vi "UMLEditor_PackageClasses.vi"(0 "DiagramIn":refnum<class "Graph.lvclass">, 3 "Settings":T1={"Levels"=-1}, 5 "error in (no error)":errorcluster) -> (19 "error out":errorcluster)   [LabVIEW 2020]
doc: "Gets current diagram values"
uses:
  <resource>/Framework/Providers/Open_GDS/UML/UMLEditor/UMLEditor_PackageClasses.ctl
  <resource>/Framework/Providers/Open_GDS/UML/Graph_class/Graph.lvclass
  <resource>/Framework/Providers/Open_GDS/UML/Graphics_class/FontType.ctl
  <resource>/Framework/Providers/Open_GDS/UML/UMLEditor/UMLEditor BusyDialogAction.ctl
  <resource>/Framework/Providers/Open_GDS/UML/ClassNode_class/ClassNode.lvclass
  C:/Program Files (x86)/National Instruments/LabVIEW 2020/resource/Framework/Providers/Open_GDS/UML/AbstractNode_class/AbstractNode.lvclass
  <resource>/Framework/Providers/Open_GDS/UML/PackageNode_class/PackageNode.lvclass
  C:/Program Files (x86)/National Instruments/LabVIEW 2020/resource/Framework/Providers/Open_GDS/UML/RectangularNode_class/RectangularNode.lvclass
  <resource>/Framework/Providers/Open_GDS/UML/ContextHelp/ContextHelp_HelpTexts.ctl
  <resource>/Framework/Providers/Open_GDS/UML/General/Point/Point Point2D.ctl
  <resource>/Framework/Providers/Open_GDS/UML/RectangularNode_class/RectangularNode.lvclass
  <resource>/Framework/Providers/Open_GDS/UML/Graphics_class/Graphics.lvclass
  <resource>/Framework/Providers/Open_GDS/UML/AbstractNode_class/AbstractNode.lvclass
panel:
  in  "MoveNodes":bool
  in  "Levels":i32=3 caption="Maximum levels of packages to create" min=1 max=100
  in  "Help":bool
  in  "cancel":bool
  in  "ok":bool
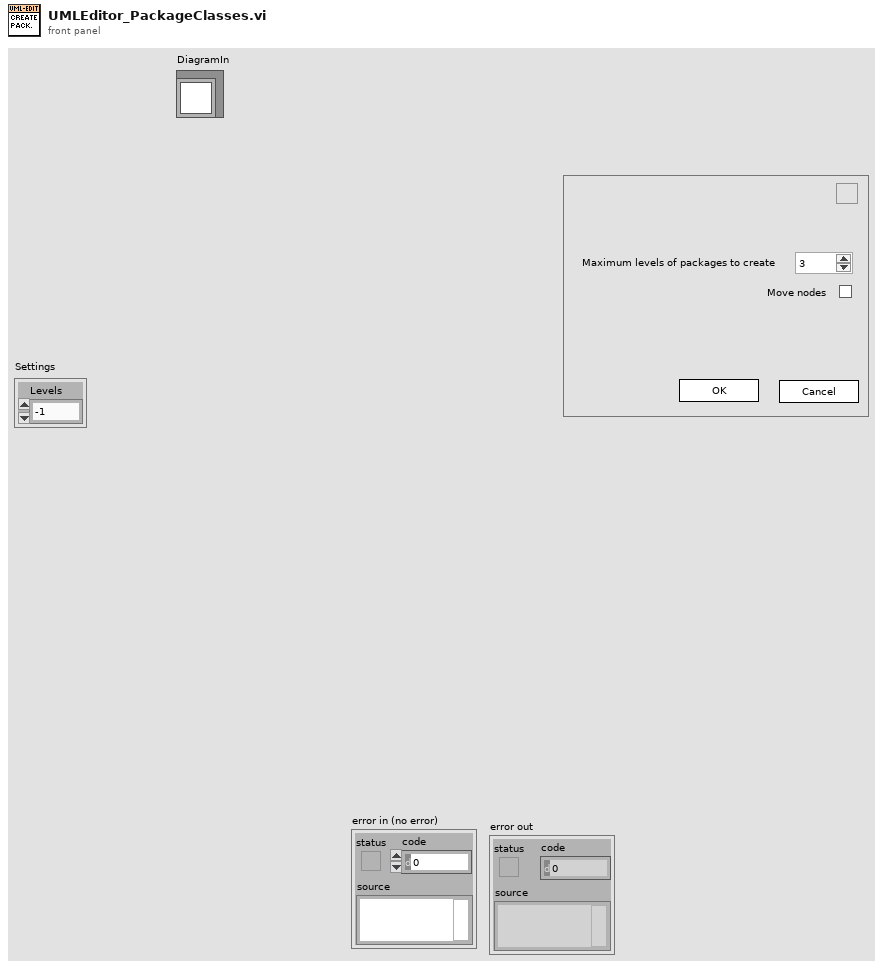
[diagram p1: front panel]
types:
  T1 = typedef "UMLEditor_PackageClasses.ctl" = cluster{"Levels":i32}
  T2 = cluster{"ClassNodes":refnum<class "ClassNode.lvclass">[], "Folders":cluster{"Foldername":string, "Path":path, "Nodes":refnum<class "ClassNode.lvclass">[], "SubFolders":path[], "PackageNode":refnum<class "PackageNode.lvclass">}[], "PackageNames":string[], "PackagesNodes":refnum<class "PackageNode.lvclass">[]}
  T3 = typedef "UMLEditor BusyDialogAction.ctl" = enum16{"Initialize", "Open(VIs)", "Open(i)", "Send_I-Value", "SendStatusMessage", "GetBusyDialogStatus", "Close", "Quit"}
  T4 = typedef "Graphics.lvclass/FontType.ctl" = cluster{"Font Name:":string, "Size":i16, "Strikeout?":bool, "Italic?":bool, "Underline?":bool, "Outline?":bool, "Shadow?":bool, "Bold?":bool}
  T5 = typedef "ContextHelp_HelpTexts.ctl" = enum16{"None(Hide)", "Default", "Help", "Welcome", "GettingStarted", "ClassDiagram_Help", "SequenceDiagram_Help", "UseCaseDiagram_Help", "BSelect", "BClass", "BInterface", "BPackage", "BNote", "BDependency", "BInheritance", "BInterfaceImplementation", "BAssociation", "BAggregation", "BCompAggregation", "BNoteConnector", "BObject", "BActionBar", "BCall", "BSystem", "BActor", "BUseCase", "BGeneralization", "BIncludes", "BExtends", "BUseCaseDiagramAssociation", "ClassRelationshipEdge editDialog_Bent Style", "ClassRelationshipEdge editDialog_RelationType", "ClassRelationshipEdge editDialog_Reverse association", "ClassRelationshipEdge editDialog_Start label", "ClassRelationshipEdge editDialog_Middle label", "ClassRelationshipEdge editDialog_End label", "UMLEditor reversedEngineering_Pathes", "ReversedEngineering StateReverseDialog_Help", "ReversedEngineering StateQueuedSettings_Help", "UMLEditor reversedEngineering_AddTopVIs", "UMLEditor reversedEngineering_AddClasses", "UMLEditor reversedEngineering_AddDirs", "UMLEditor reversedEngineering_Recursively", "UMLEditor reversedEngineering_Remove", "UMLEditor reversedEngineering_ClearList", "UMLEditor reversedEngineering_HideSubAss", "UMLEditor reversedEngineering_CreateTypes", "UMLEditor reversedEngineering_OnlyInheritance", "UMLEditor reversedEngineering_CreateApplication", "UMLEditor reversedEngineering_OK", "UMLEditor reversedEngineering_Cancel", "UMLEditor reversedEngineering_Help", "UMLEditor createWizardScriptFile_ScriptfilePath", "UMLEditor createWizardScriptFile_ClassPath", "UMLEditor createWizardScriptFile_Use", "UMLEditor createWizardScriptFile_PrivateDirName", "UMLEditor createWizardScriptFile_DirAppend", "UMLEditor createWizardScriptFile_Separator Character", "UMLEditor createWizardScriptFile_OK", "UMLEditor createWizardScriptFile_Cancel", "UMLEditor createWizardScriptFile_Help", "ClassNode editDialog_Class Name", "InterfaceNode editDialog_Class Name", "ClassNode editDialog_Attribute", "ClassNode editDialog_Methods", "InterfaceNode editDialog_Methods", "ClassNode editDialog_connection", "InterfaceNode editDialog_connection", "ClassNode editDialog_StereoType", "ClassNode editDialog_ShowAttrib", "ClassNode editDialog_ShowMethods", "ClassNode editDialog_ClassPath", "ClassNode editDialog_AddAttribute", "ClassNode editDialog_AddMethod", "InterfaceNode editDialog_AddMethod", "ClassNode AttributeGuide_AttributeName", "ClassNode AttributeGuide_Array?", "ClassNode AttributeGuide_Data Type", "ClassNode AttributeGuide_RefName", "ClassNode AttributeGuide_Preview", "ClassNode AttributeGuide_OK", "ClassNode AttributeGuide_Cancel", "ClassNode MethodGuide_Visibility", "ClassNode MethodGuide_Method Name", "ClassNode MethodGuide_Preview", "ClassNode MethodGuide_OK", "ClassNode MethodGuide_Cancel", "CallNode EditCallProperties_AllButtons", "ObjectNode EditObjectlProperties_AllButtons", "ActorNode EditActorProperties_AllButtons", "UseCaseRelationshipNode EditUseCaselProperties_AllButtons", "UseCaseNode EditUseCaselProperties_AllButtons", "SystemNode EditSystemProperties_AllButtons", "ReversedEngineering UpdateAttributes_AllButtons", "StateNode editDialog_AllButtons", "StateTransition editDialog_AllButtons", "ArrangeNodes Main_Picture", "ArrangeNodes Main_Zoom", "ArrangeNodes Main_Auto Zoom", "ArrangeNodes Main_shorten", "ArrangeNodes Main_Min Length", "ArrangeNodes Main_Max Length", "ArrangeNodes Main_increase", "ArrangeNodes Main_decrease", "ArrangeNodes Main_Shake", "ArrangeNodes Main", "BState", "BInitialState", "BFinalState", "BStateTransition", "StateDiagram_Help", "StateDiagram_PropertiesAllButtons", "ReversedEngineering StateReverseDialog_ClearStates", "ReversedEngineering StateReverseDialog_UseQueuedStateMachines", "ReversedEngineering StateReverseDialog_QueuedSettings", "ReversedEngineering StateReverseDialog_SearchForVIs", "ReversedEngineering StateReverseDialog_SearchCriteria", "OptionsDialog_ClassBasePath", "OptionsDialog_VIPath", "OptionsDialog_ApplicationPath", "OptionsDialog_WizDir", "OptionsDialog_IniFilePath", "OptionsDialog_DefineColors", "OptionsDialog_Help", "OptionsDialog_CreateTypes", "ClassRelationshipEdge editDialog_SplitWire"}
  T6 = typedef "Point Point2D.ctl" = cluster{"x":dbl, "y":dbl}
  T7 = typedef "ContextHelp_ShowType.ctl" = cluster{"Header":string, "Picture":picture, "Text":string}
  T8 = cluster{"Foldername":string, "Path":path, "Nodes":refnum<class "ClassNode.lvclass">[], "SubFolders":path[], "PackageNode":refnum<class "PackageNode.lvclass">}
  T9 = cluster{"Foldername":string, "Path":path, "Nodes":refnum<class "ClassNode.lvclass">[], "SubFolders":path[], "PackageNode":refnum<class "PackageNode.lvclass">}[]
  T10 = typedef "Rectangle Rectangle2D.ctl" = cluster{"x":dbl, "y":dbl, "width":dbl, "height":dbl}
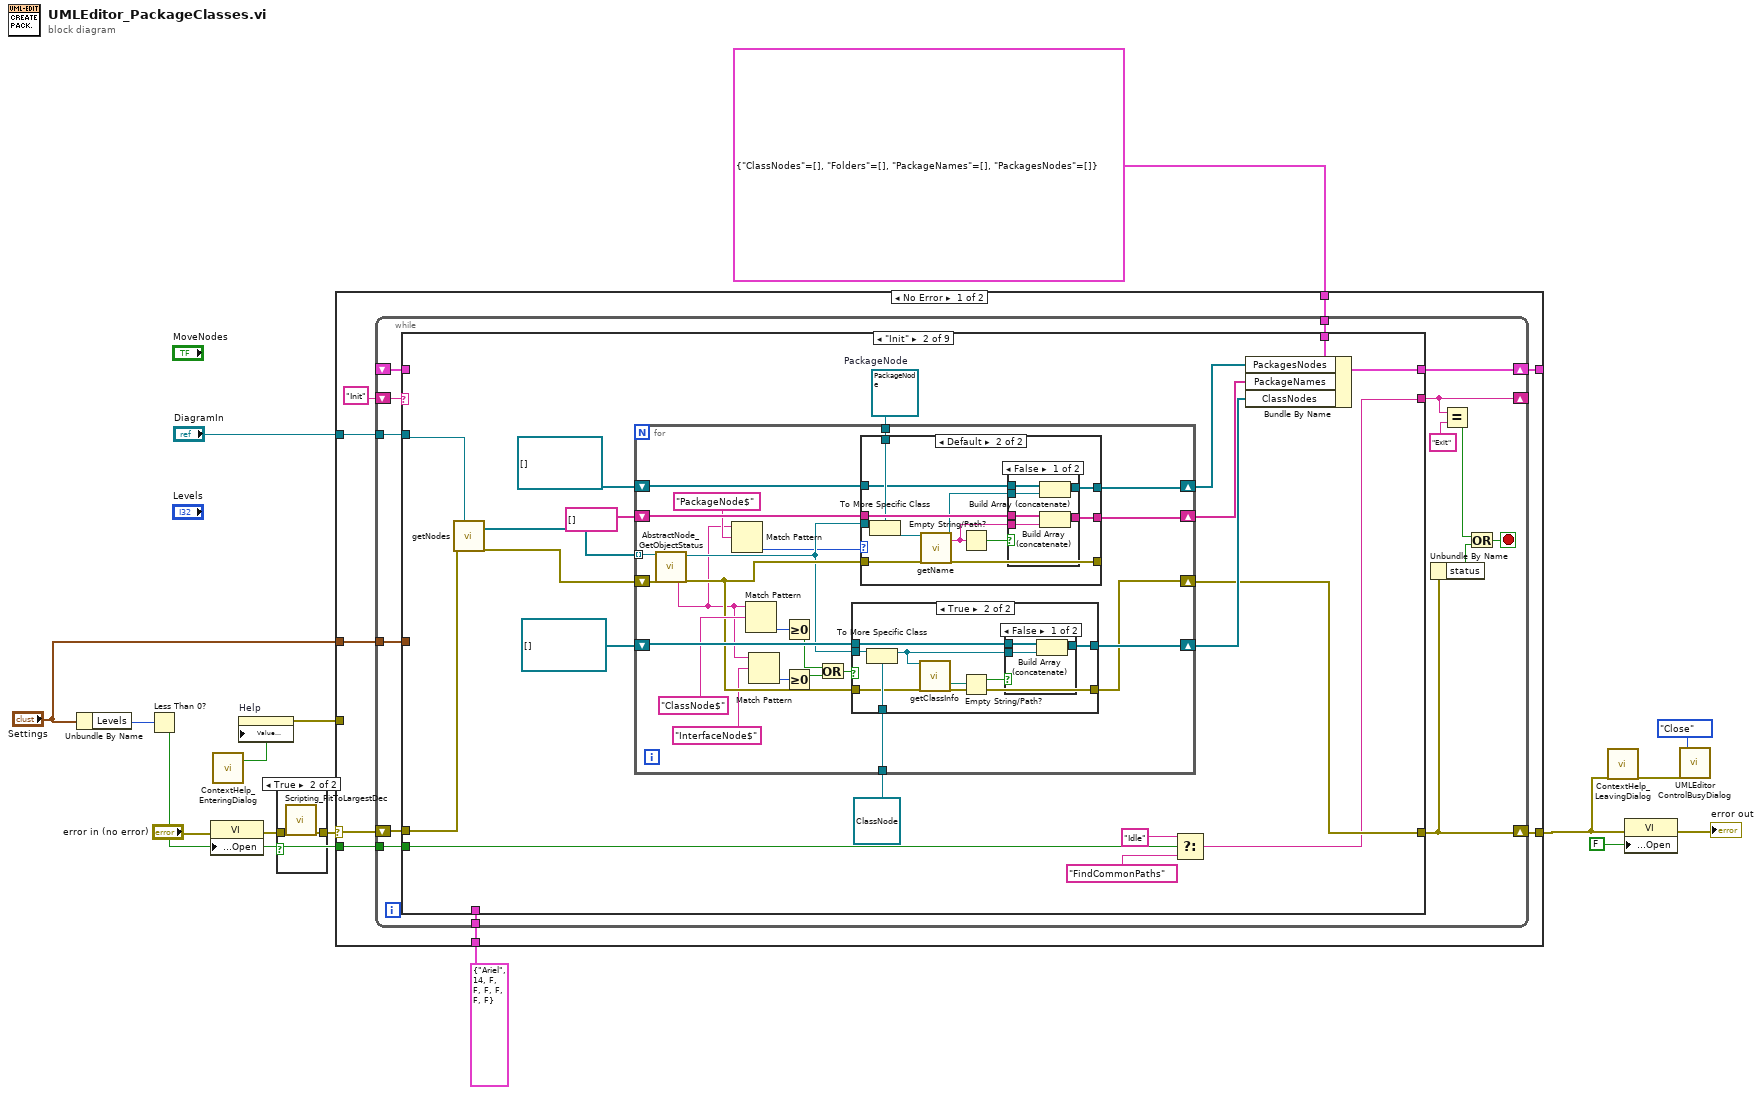
[diagram p0: block diagram]
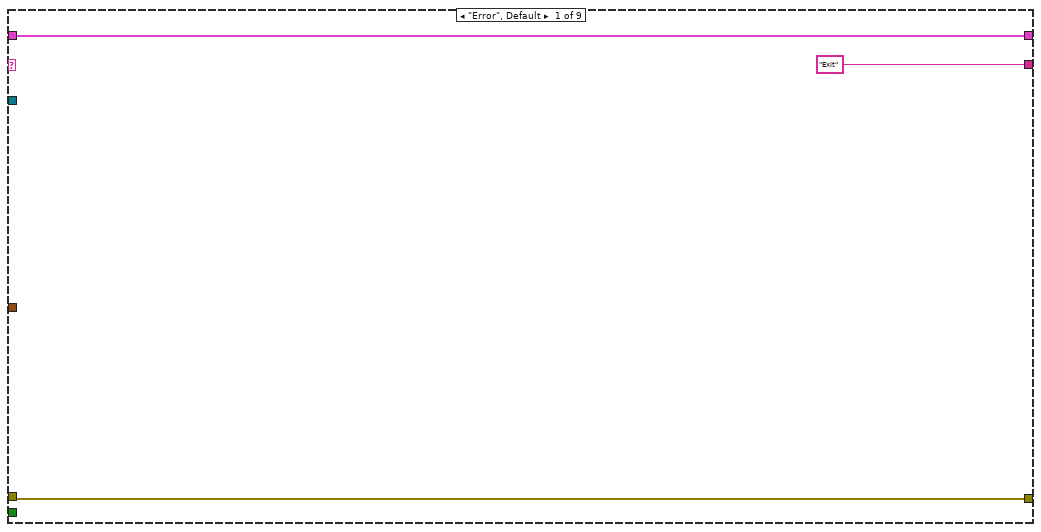
[diagram p3: hidden frame]
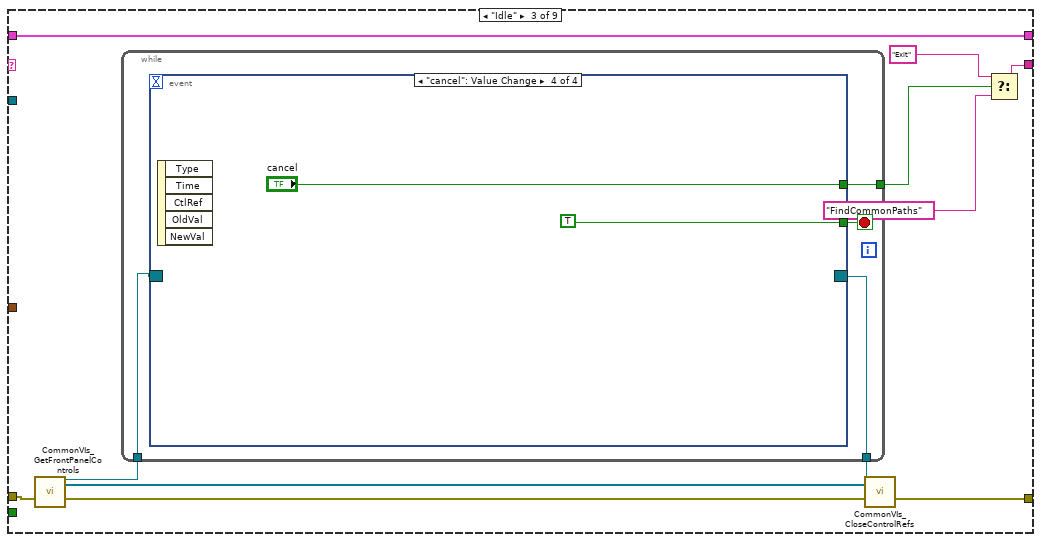
[diagram p8: hidden frame]
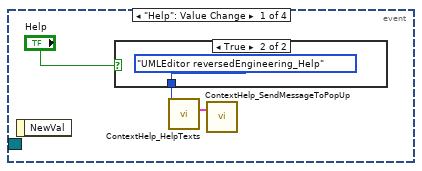
[diagram p9: hidden frame]
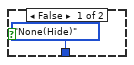
[diagram p10: hidden frame]
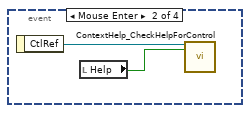
[diagram p11: hidden frame]
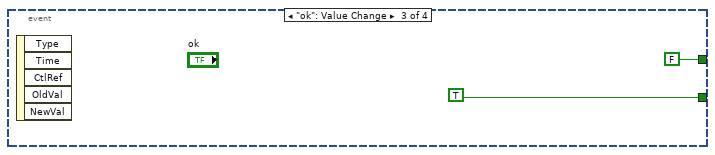
[diagram p12: hidden frame]
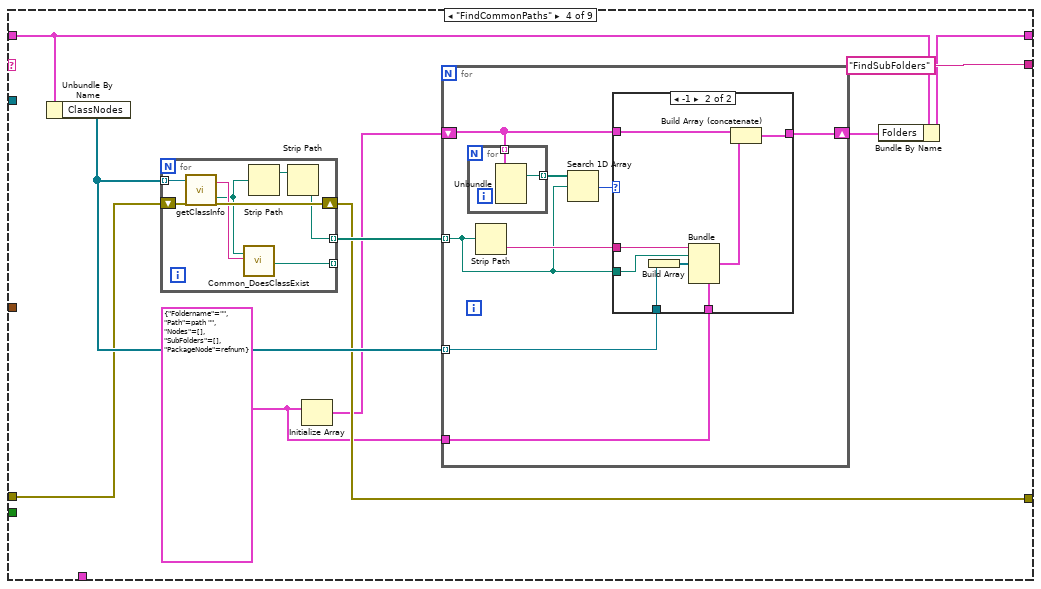
[diagram p13: hidden frame]
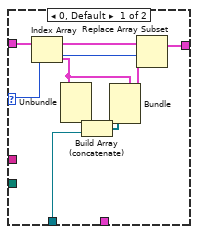
[diagram p14: hidden frame]
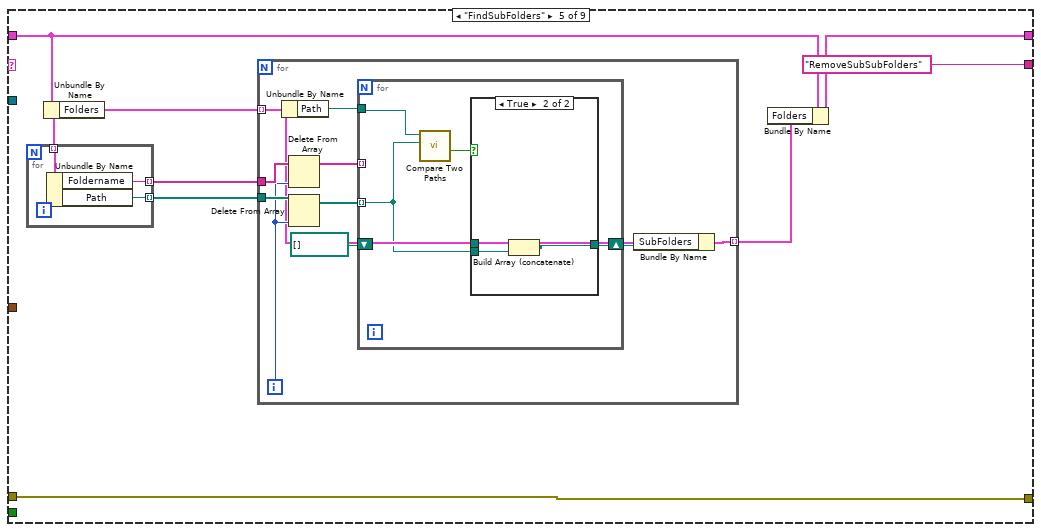
[diagram p15: hidden frame]
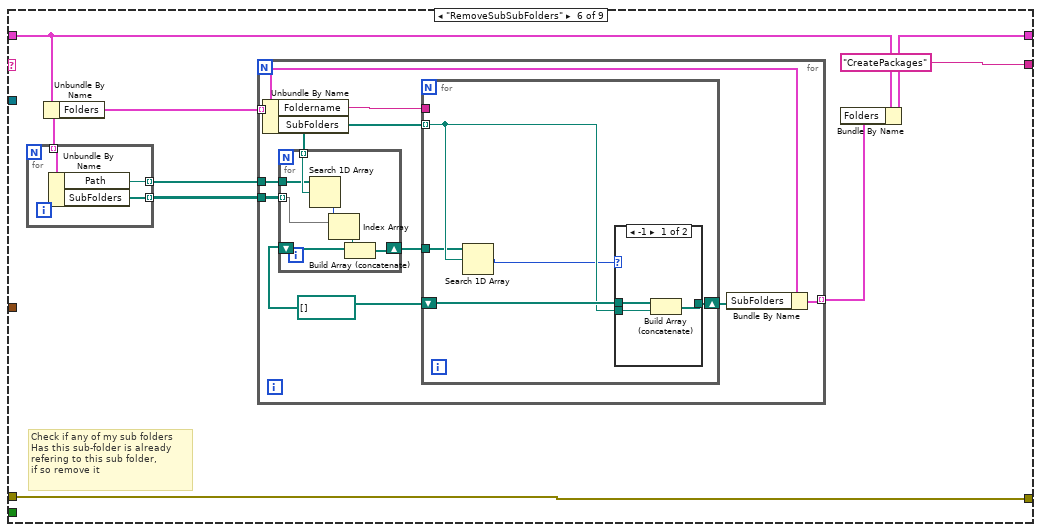
[diagram p17: hidden frame]
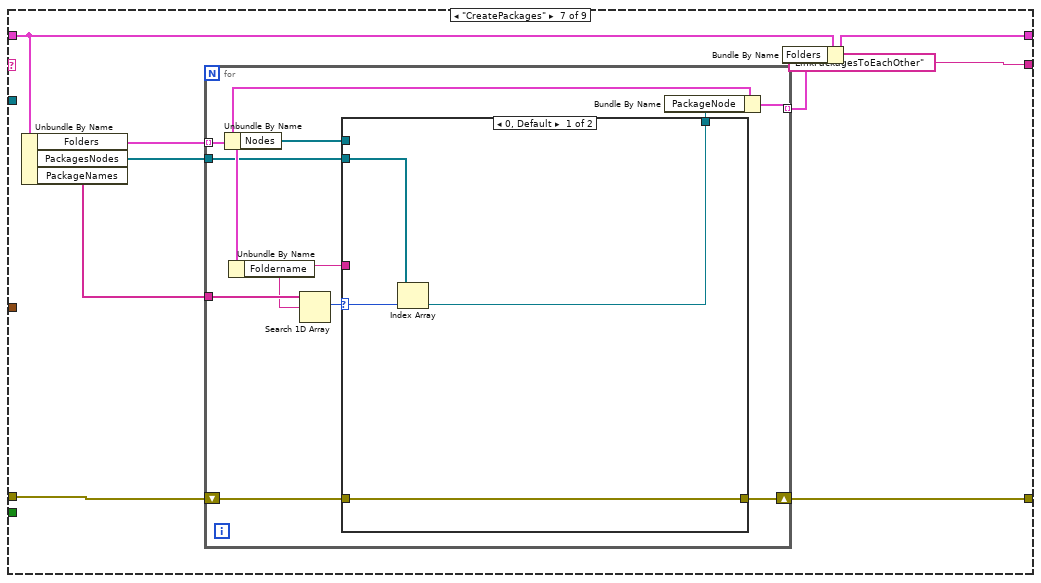
[diagram p19: hidden frame]
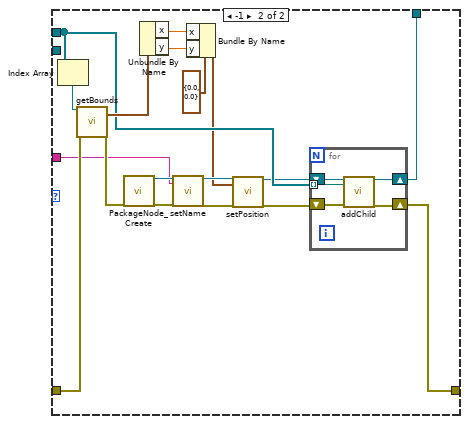
[diagram p20: hidden frame]
diagram:
  n1 = Unbundle By Name("Settings") -> ("Levels"=w5:i32)
  n2 = Less Than 0?(x=w5) -> (x < 0?=w4:bool)
  n3 = property class="VI"(error in="error in (no error)", "Front Panel.Open"=w4) -> (error out=w7:errorcluster)  [unwired: 1 in, 1 out]
  n4 = call <resource>:"ContextHelp_EnteringDialog.vi"() -> ("HelpStatus"=w16:bool)  [unwired: 1 in, 18 out]
  n5 = property on="Help" class="Bool (strict)"("Value (Signaling)"=w16) -> (error out=w15:errorcluster)  [unwired: 2 in, 1 out]
  n6 = case shown="True" w4 {
    tunnel: w7 -> [w17 w19]
    tunnel: [w17 w18] -> w6
    frame False {
    }
    frame True {
      n7 = call <resource>:"Scripting_FitToLargestDec.vi"("error in (no error)"=w19) -> ("error out"=w18:errorcluster)  [unwired: 5 in, 1 out]
    }
  }
  n8 = case shown="No Error" w6 {
    selector: w6 -> [w26 w379]
    tunnel: [w27 w379] -> w12
    tunnel: [w25 _] -> _
    tunnel: w15 -> [_ _]
    tunnel: T4 {"Font Name:"="Ariel", "Size"=14, "Strikeout?"=FALSE, "Italic?"=FALSE, "Underline?"=FALSE, "Outline?"=FALSE, "Shadow?"=FALSE, "Bold?"=FALSE} ("font") -> [w24 _]
    tunnel: w4 -> [w23 _]
    tunnel: T2 {"ClassNodes"=[], "Folders"=[], "PackageNames"=[], "PackagesNodes"=[]} ("local") -> [w22 _]
    tunnel: "Settings" -> [w21 _]
    tunnel: "DiagramIn" -> [w20 _]
    frame No Error {
      n9 = while {
        shift-right: [w40] -> w27
        shift-left: w26 -> [w29]
        shift-right: [w38] -> _
        shift-left: "Init" -> [w43]
        shift-right: [w42] -> w25
        shift-left: _ -> [w41]
        tunnel: w24 -> [w34]
        tunnel: w23 -> [w33]
        tunnel: w22 -> [w32]
        tunnel: w21 -> [w31]
        tunnel: w20 -> [w30]
        stop <- w35 stop-if-true
        n10 = case shown="\"Init\"" w43 {
          tunnel: [w44 w57 w127 w158 w201 w232 w264 w309 w355] -> w40
          tunnel: [w45 w60 w129 w153 w195 w226 w265 w314 w359] -> w42
          tunnel: ["Exit" w53 w134 "FindSubFolders" ("y") "RemoveSubSubFolders" ("y") "CreatePackages" ("y") "LinkPackagesToEachOther" ("y") "AddPackagesToGraph" ("y") "Exit" ("y")] -> w38
          tunnel: w41 -> [w45 _ w129 w154 w196 w227 w266 w314 w359]
          tunnel: w34 -> [_ _ _ _ _ _ _ _ _]
          tunnel: w33 -> [_ w56 _ _ _ _ _ _ _]
          tunnel: w32 -> [_ w61 _ _ _ _ _ _ _]
          tunnel: w31 -> [_ _ _ _ _ _ _ _ _]
          tunnel: w30 -> [_ w62 _ _ _ _ _ _ w360]
          tunnel: w29 -> [w44 w51 w127 w152 w201 w232 w263 w315 w354]
          frame "Error", Default {
          }
          frame "Init" {
            w50 = refnum<class "PackageNode.lvclass"> refnum  # PackageNode
            n11 = call-dynamic "getNodes.vi"("reference"=w62, "error in (no error)"=w51) -> ("nodes"=w59:refnum<class "AbstractNode.lvclass">[], "error out"=w64:errorcluster)  [unwired: 15 in, 1 out]
            n12 = for {
              shift-right: [w82] -> w57
              shift-left: w64 -> [w88]
              tunnel: w59 -> [w87] mode=indexing
              shift-right: [w85] -> w58
              shift-left: refnum<class "ClassNode.lvclass">[] [] -> [w86]
              tunnel: refnum<class "ClassNode.lvclass"> refnum ("reference out") -> [w83]
              shift-right: [w75] -> w49
              shift-left: string[] [] -> [w79]
              tunnel: w50 -> [w81]
              shift-right: [w74] -> w47
              shift-left: refnum<class "PackageNode.lvclass">[] [] -> [w73]
              n13 = call <resource>:"AbstractNode_GetObjectStatus.vi"("reference in"=w87, "error in (no error)"=w88) -> ("Class name"=w72:string, "reference out"=w78:refnum<class "AbstractNode.lvclass">, "error out"=w80:errorcluster)  [unwired: 15 out]
              n14 = Match Pattern(string=w72, regular expression="PackageNode$") -> (offset past match=w76:i32)  [unwired: 4 out]
              n15 = Match Pattern(string=w72, regular expression="ClassNode$") -> (offset past match=w69:i32)  [unwired: 4 out]
              n16 = Match Pattern(string=w72, regular expression="InterfaceNode$") -> (offset past match=w70:i32)  [unwired: 4 out]
              n17 = Greater Or Equal To 0?(x=w69) -> (x >= 0?=w67:bool)
              n18 = Greater Or Equal To 0?(x=w70) -> (x >= 0?=w68:bool)
              n19 = Or(x=w67, y=w68) -> (x .or. y?=w66:bool)
              n20 = case shown="True" w66 {
                tunnel: w86 -> [w113 w122]
                tunnel: w78 -> [_ w120]
                tunnel: [w113 w121] -> w85
                tunnel: w83 -> [_ w119]
                tunnel: w80 -> [w112 w117]
                tunnel: [w112 w114] -> w82
                frame False {
                }
                frame True {
                  n21 = To More Specific Class(target class=w119, reference=w120) -> (specific class reference=w118:refnum<class "ClassNode.lvclass">)  [unwired: 1 in, 1 out]
                  n22 = call-dynamic "getClassInfo.vi"("reference"=w118, "error in (no error)"=w117) -> ("ClassPath"=w116:path, "error out"=w114:errorcluster)  [unwired: 8 in, 8 out]
                  n23 = Empty String/Path?(string/path=w116) -> (empty?=w115:bool)
                  n24 = case shown="False" w115 {
                    tunnel: w122 -> [w125 w126]
                    tunnel: [w124 w126] -> w121
                    tunnel: w118 -> [w123 _]
                    frame False {
                      n25 = Build Array (concatenate)(w125, w123) -> (w124:refnum<class "ClassNode.lvclass">[])
                    }
                    frame True {
                    }
                  }
                }
              }
              n26 = case shown="Default" w76 {
                tunnel: w79 -> [w91 w103]
                tunnel: w78 -> [_ w101]
                tunnel: [w91 w102] -> w75
                tunnel: w80 -> [w90 w97]
                tunnel: [w90 w95] -> _
                tunnel: w81 -> [_ w99]
                tunnel: [w89 w94] -> w74
                tunnel: w73 -> [w89 w93]
                frame -1 {
                }
                frame Default {
                  n27 = To More Specific Class(target class=w99, reference=w101) -> (specific class reference=w98:refnum<class "PackageNode.lvclass">)  [unwired: 1 in, 1 out]
                  n28 = call-dynamic "getName.vi"("reference"=w98, "error in (no error)"=w97) -> ("reference out"=w92:refnum<class "PackageNode.lvclass">, "name"=w96:string, "error out"=w95:errorcluster)  [unwired: 15 in]
                  n29 = Empty String/Path?(string/path=w96) -> (empty?=w100:bool)
                  n30 = case shown="False" w100 {
                    tunnel: w103 -> [w106 w111]
                    tunnel: [w109 w111] -> w102
                    tunnel: w96 -> [w108 _]
                    tunnel: [w107 w110] -> w94
                    tunnel: w93 -> [w105 w110]
                    tunnel: w92 -> [w104 _]
                    frame False {
                      n31 = Build Array (concatenate)(w105, w104) -> (w107:refnum<class "PackageNode.lvclass">[])
                      n32 = Build Array (concatenate)(w106, w108) -> (w109:string[])
                    }
                    frame True {
                    }
                  }
                }
              }
            }
            n33 = Select(t="Idle" ("y"), s=w56, f="FindCommonPaths") -> (s? t:f=w53:string)
            n34 = Bundle By Name(cluster=w61, "PackagesNodes"=w47, "PackageNames"=w49, "ClassNodes"=w58) -> (w60:T2)
          }
          frame "Idle" {
            n35 = call <resource>:"CommonVIs_GetFrontPanelControls.vi"() -> ("Event Registration Refnum"=w132:refnum<event-registration>, "ControlRefs"=w130:refnum<vi>[])  [unwired: 2 in, 16 out]
            n36 = while {
              tunnel: [w139] -> w128
              tunnel: w132 -> [w137]
              tunnel: [w136] -> w131
              stop <- w138 stop-if-true
              n37 = event shown="[3] \"cancel\": Value Change" {
                selector: w137 -> [_ _ _ _]
                dyn-events: [_ _ _ _] -> w136
                timeout: _ -> [_ _ _ _]
                tunnel: [_ _ FALSE ("cancel") "cancel"] -> w139
                tunnel: [_ _ TRUE ("Front Panel Window:Is Frontmost") TRUE ("Front Panel Window:Is Frontmost")] -> w138
                event "Help": Value Change {
                  n38 = event-data() -> ()  [unwired: 2 out]
                  n39 = case shown="True" "Help" {
                    tunnel: [ContextHelp_HelpTexts."None(Hide)" ("HelpText") ContextHelp_HelpTexts."UMLEditor reversedEngineering_Help" ("HelpText")] -> w141
                    frame False {
                    }
                    frame True {
                    }
                  }
                  n40 = call <resource>:"ContextHelp_HelpTexts.vi"("HelpText (enum or string)"=w141) -> ("HelpOut"=w142:T7)  [unwired: 18 out]
                  n41 = call <resource>:"ContextHelp_SendMessageToPopUp.vi"("PopUpMessage"=w142) -> ()  [unwired: 2 in, 17 out]
                }
                event Mouse Enter {
                  n42 = event-data() -> ("CtlRef"=w146:refnum<vi>)  [unwired: 1 out]
                  n43 = local read "Help"() -> (w145:bool)
                  n44 = call <resource>:"ContextHelp_CheckHelpForControl.vi"("Ctl Refnum"=w146, "Help"=w145) -> ()  [unwired: 1 in, 17 out]
                }
                event "ok": Value Change {
                  n45 = event-data() -> ()  [unwired: 6 out]
                }
                event "cancel": Value Change {
                  n46 = event-data() -> ()  [unwired: 6 out]
                }
              }
            }
            n47 = call <resource>:"CommonVIs_CloseControlRefs.vi"("Event Registration Refnum"=w131, "ControlRefs"=w130) -> ()  [unwired: 1 in, 17 out]
            n48 = Select(t="Exit", s=w128, f="FindCommonPaths") -> (s? t:f=w134:string)
          }
          frame "FindCommonPaths" {
            w156 = T8 {"Foldername"="", "Path"=path "", "Nodes"=[], "SubFolders"=[], "PackageNode"=refnum}
            n49 = Unbundle By Name(w154) -> ("ClassNodes"=w160:refnum<class "ClassNode.lvclass">[])
            n50 = for {
              tunnel: w160 -> [w194] mode=indexing
              shift-right: [w192] -> w158
              shift-left: w152 -> [w193]
              tunnel: [w187] -> w159 mode=indexing
              tunnel: [w190] -> _ mode=indexing
              n51 = call-dynamic "getClassInfo.vi"("reference"=w194, "error in (no error)"=w193) -> ("className"=w191:string, "ClassPath"=w188:path, "error out"=w192:errorcluster)  [unwired: 8 in, 7 out]
              n52 = call <resource>:"Common_DoesClassExist.vi"("ClassPath"=w188, "ClassName"=w191) -> ("llb/LvCLass-Path"=w190:path)  [unwired: 17 out]
              n53 = Strip Path(path=w188) -> (stripped path=w189:path)  [unwired: 1 out]
              n54 = Strip Path(path=w189) -> (stripped path=w187:path)  [unwired: 1 out]
            }
            n55 = Initialize Array(w156) -> (w157:T9)  [unwired: 1 in]
            n56 = for {
              tunnel: w159 -> [w161] mode=indexing
              tunnel: w160 -> [w163] mode=indexing
              shift-right: [w168] -> w151
              shift-left: w157 -> [w166]
              tunnel: w156 -> [w162]
              n57 = for {
                tunnel: [w185] -> w167 mode=indexing
                tunnel: w166 -> [w186] mode=indexing
                n58 = Unbundle(w186) -> ("Path"=w185:path)  [unwired: 4 out]
              }
              n59 = Strip Path(path=w161) -> (name=w165:string)  [unwired: 1 out]
              n60 = Search 1D Array(1D array=w167, element=w161) -> (index of element=w164:i32)  [unwired: 1 in]
              n61 = case shown="-1" w164 {
                selector: w164 -> [w173 _]
                tunnel: w161 -> [_ w184]
                tunnel: [w172 w183] -> w168
                tunnel: w166 -> [w174 w182]
                tunnel: w165 -> [_ w181]
                tunnel: w163 -> [w175 w180]
                tunnel: w162 -> [_ w179]
                frame 0, Default {
                  n62 = Index Array(array=w174, index=w173) -> (element=w171:T8)
                  n63 = Unbundle(w171) -> ("Nodes"=w176:refnum<class "ClassNode.lvclass">[])  [unwired: 4 out]
                  n64 = Build Array (concatenate)(w176, w175) -> (w170:refnum<class "ClassNode.lvclass">[])
                  n65 = Bundle(cluster=w171, "Nodes"=w170) -> (w169:T8)  [unwired: 4 in]
                  n66 = Replace Array Subset(array=w174, new element=w169, index=w173) -> (w172:T9)
                }
                frame -1 {
                  n67 = Build Array(w180) -> (w178:refnum<class "ClassNode.lvclass">[])
                  n68 = Bundle(cluster=w179, "Foldername"=w181, "Path"=w184, "Nodes"=w178) -> (w177:T8)  [unwired: 2 in]
                  n69 = Build Array (concatenate)(w182, w177) -> (w183:T9)
                }
              }
            }
            n70 = Bundle By Name(cluster=w154, "Folders"=w151) -> (w153:T2)
          }
          frame "FindSubFolders" {
            n71 = Unbundle By Name(w196) -> ("Folders"=w200:T9)
            n72 = for {
              tunnel: w200 -> [w205] mode=indexing
              tunnel: [w204] -> w198 mode=indexing
              tunnel: [w203] -> w199 mode=indexing
              n73 = Unbundle By Name(w205) -> ("Foldername"=w204:string, "Path"=w203:path)
            }
            n74 = for {
              tunnel: w200 -> [w209] mode=indexing
              tunnel: w199 -> [w215]
              tunnel: w198 -> [w214]
              tunnel: [w207] -> w197 mode=indexing
              i -> [w213]
              n75 = Unbundle By Name(w209) -> ("Path"=w212:path)
              n76 = Delete From Array(array=w214, index=w213) -> (array with subset deleted=w210:string[])  [unwired: 1 in, 1 out]
              n77 = Delete From Array(array=w215, index=w213) -> (array with subset deleted=w211:path[])  [unwired: 1 in, 1 out]
              n78 = for {
                tunnel: w212 -> [w220]
                tunnel: w211 -> [w216] mode=indexing
                shift-right: [w217] -> w208
                shift-left: path[] [] -> [w218]
                tunnel: w210 -> [_] mode=indexing
                n79 = call <vilib>:"Compare Two Paths.vi"("Path 2"=w216, "Path 1"=w220) -> ("Path 2 Relative to Path 1?"=w219:bool)  [unwired: 6 in, 3 out]
                n80 = case shown="True" w219 {
                  tunnel: w218 -> [w221 w224]
                  tunnel: w216 -> [_ w223]
                  tunnel: [w221 w222] -> w217
                  frame False {
                  }
                  frame True {
                    n81 = Build Array (concatenate)(w224, w223) -> (w222:path[])
                  }
                }
              }
              n82 = Bundle By Name(cluster=w209, "SubFolders"=w208) -> (w207:T8)
            }
            n83 = Bundle By Name(cluster=w196, "Folders"=w197) -> (w195:T2)
          }
          frame "RemoveSubSubFolders" {
            # "Check if any of my sub folders\nHas this sub-folder is already \nrefering to this sub folder,\nif so remove it"
            n84 = Unbundle By Name(w227) -> ("Folders"=w231:T9)
            n85 = for {
              tunnel: w231 -> [w235] mode=indexing
              tunnel: [w234] -> w229 mode=indexing
              tunnel: [w233] -> w230 mode=indexing
              n86 = Unbundle By Name(w235) -> ("Path"=w234:path, "SubFolders"=w233:path[])
            }
            n87 = for {
              tunnel: w231 -> [w243] mode=indexing
              tunnel: w230 -> [w238]
              tunnel: w229 -> [w240]
              tunnel: [w241] -> w228 mode=indexing
              w237 = path[] []
              n88 = Unbundle By Name(w243) -> ("Foldername"=w244:string, "SubFolders"=w239:path[])
              n89 = for {
                tunnel: w239 -> [w251] mode=indexing
                tunnel: w240 -> [w245]
                tunnel: w238 -> [w250] mode=indexing
                shift-right: [w246] -> w236
                shift-left: w237 -> [w248]
                n90 = Search 1D Array(1D array=w245, element=w251) -> (index of element=w249:i32)  [unwired: 1 in]
                n91 = Index Array(array=w250, index=w249) -> (element=w247:path)
                n92 = Build Array (concatenate)(w248, w247) -> (w246:path[])
              }
              n93 = for {
                tunnel: w244 -> [_]
                shift-right: [w255] -> w242
                shift-left: w237 -> [w256]
                tunnel: w239 -> [w254] mode=indexing
                tunnel: w236 -> [w253]
                n94 = Search 1D Array(1D array=w253, element=w254) -> (index of element=w252:i32)  [unwired: 1 in]
                n95 = case shown="-1" w252 {
                  tunnel: w256 -> [w259 w260]
                  tunnel: [w258 w260] -> w255
                  tunnel: w254 -> [w257 _]
                  frame -1 {
                    n96 = Build Array (concatenate)(w259, w257) -> (w258:path[])
                  }
                  frame Default {
                  }
                }
              }
              n97 = Bundle By Name(cluster=w243, "SubFolders"=w242) -> (w241:T8)
            }
            n98 = Bundle By Name(cluster=w227, "Folders"=w228) -> (w226:T2)
          }
          frame "CreatePackages" {
            n99 = Unbundle By Name(w266) -> ("Folders"=w268:T9, "PackagesNodes"=w261:refnum<class "PackageNode.lvclass">[], "PackageNames"=w262:string[])
            n100 = for {
              tunnel: w268 -> [w277] mode=indexing
              shift-right: [w275] -> w264
              shift-left: w263 -> [w279]
              tunnel: [w274] -> w267 mode=indexing
              tunnel: w262 -> [w273]
              tunnel: w261 -> [w270]
              n101 = Unbundle By Name(w277) -> ("Nodes"=w278:refnum<class "ClassNode.lvclass">[])
              n102 = Unbundle By Name(w277) -> ("Foldername"=w272:string)
              n103 = Search 1D Array(1D array=w273, element=w272) -> (index of element=w271:i32)  [unwired: 1 in]
              n104 = case shown="0, Default" w271 {
                selector: w271 -> [w282 _]
                tunnel: w279 -> [w283 w298]
                tunnel: w278 -> [_ w292]
                tunnel: [w280 w286] -> w276
                tunnel: [w283 w285] -> w275
                tunnel: w272 -> [_ w284]
                tunnel: w270 -> [w281 _]
                frame 0, Default {
                  n105 = Index Array(array=w281, index=w282) -> (element=w280:refnum<class "PackageNode.lvclass">)
                }
                frame -1 {
                  n106 = Index Array(array=w292) -> (element=w299:refnum<class "ClassNode.lvclass">)  [unwired: 1 in]
                  n107 = call-dynamic "getBounds.vi"("reference"=w299, "error in (no error)"=w298) -> ("bounds"=w296:T10, "error out"=w297:errorcluster)  [unwired: 15 in, 1 out]
                  n108 = call <resource>:"PackageNode_Create.vi"("error in (no error)"=w297) -> ("reference out"=w301:refnum<class "PackageNode.lvclass">, "error out"=w300:errorcluster)  [unwired: 17 in]
                  n109 = Unbundle By Name(w296) -> ("x"=w294:dbl, "y"=w293:dbl)
                  n110 = call-dynamic "setName.vi"("reference"=w301, "name"=w284, "error in (no error)"=w300) -> ("reference out"=w290:refnum<class "PackageNode.lvclass">, "error out"=w291:errorcluster)  [unwired: 15 in]
                  n111 = Bundle By Name(cluster=T6 {"x"=0.0, "y"=0.0} ("point"), "x"=w294, "y"=w293) -> (w287:T6)
                  n112 = call <resource>:"setPosition.vi"("reference"=w290, "pos"=w287, "error in (no error)"=w291) -> ("reference out"=w289:refnum<class "PackageNode.lvclass">, "error out"=w288:errorcluster)  [unwired: 2 in, 13 out]
                  n113 = for {
                    shift-right: [w305] -> w285
                    shift-left: w288 -> [w306]
                    shift-right: [w303] -> w286
                    shift-left: w289 -> [w304]
                    tunnel: w292 -> [w302] mode=indexing
                    n114 = call-dynamic "addChild.vi"("reference"=w304, "node"=w302, "error in (no error)"=w306) -> ("reference out"=w303:refnum<class "PackageNode.lvclass">, "error out"=w305:errorcluster)  [unwired: 15 in]
                  }
                }
              }
              n115 = Bundle By Name(cluster=w277, "PackageNode"=w276) -> (w274:T8)
            }
            n116 = Bundle By Name(cluster=w266, "Folders"=w267) -> (w265:T2)
          }
          frame "LinkPackagesToEachOther" {
            n117 = Unbundle By Name(w314) -> ("Folders"=w313:T9)
            n118 = for {
              tunnel: w313 -> [w326] mode=indexing
              tunnel: [w325] -> w312 mode=indexing
              tunnel: [w324] -> w311 mode=indexing
              n119 = Unbundle By Name(w326) -> ("Path"=w325:path, "PackageNode"=w324:refnum<class "PackageNode.lvclass">)
            }
            n120 = for {
              tunnel: w313 -> [w336] mode=indexing
              shift-right: [w335] -> w310
              shift-left: w315 -> [w329]
              tunnel: w312 -> [w334]
              tunnel: w311 -> [w332]
              tunnel: [w327] -> w308 mode=indexing
              i -> [w333]
              n121 = Unbundle By Name(w336) -> ("PackageNode"=w327:refnum<class "PackageNode.lvclass">)
              n122 = Unbundle By Name(w336) -> ("SubFolders"=w331:path[])
              n123 = Delete From Array(array=w334, index=w333) -> (array with subset deleted=w330:path[])  [unwired: 1 in, 1 out]
              n124 = Delete From Array(array=w332, index=w333) -> (array with subset deleted=w328:refnum<class "PackageNode.lvclass">[])  [unwired: 1 in, 1 out]
              n125 = for {
                shift-right: [w342] -> w335
                shift-left: w329 -> [w343]
                tunnel: w331 -> [w340] mode=indexing
                tunnel: w330 -> [w341]
                tunnel: w328 -> [w338]
                tunnel: w327 -> [w337]
                n126 = Search 1D Array(1D array=w341, element=w340) -> (index of element=w339:i32)  [unwired: 1 in]
                n127 = case shown="Default" w339 {
                  selector: w339 -> [w345 _]
                  tunnel: w343 -> [w350 w351]
                  tunnel: [w349 w351] -> w342
                  tunnel: w337 -> [w348 w352]
                  tunnel: [w347 w352] -> _
                  tunnel: w338 -> [w346 _]
                  frame Default {
                    n128 = Index Array(array=w346, index=w345) -> (element=w344:refnum<class "PackageNode.lvclass">)
                    n129 = call-dynamic "addChild.vi"("reference"=w348, "node"=w344, "error in (no error)"=w350) -> ("reference out"=w347:refnum<class "PackageNode.lvclass">, "error out"=w349:errorcluster)  [unwired: 15 in]
                  }
                  frame -1 {
                  }
                }
              }
            }
            n130 = for {
              N: 10 -> [_]
              tunnel: w308 -> [w317]
              shift-right: [w318] -> w309
              shift-left: w310 -> [w319]
              n131 = for {
                tunnel: w317 -> [w320] mode=indexing
                shift-right: [w321] -> w318
                shift-left: w319 -> [w322]
                n132 = call-dynamic "ExecuteMenuCommand.vi"("reference"=w320, "Command"="Size to fit", "error in (no error)"=w322) -> ("error out"=w321:errorcluster)  [unwired: 13 in, 3 out]
              }
            }
          }
          frame "AddPackagesToGraph" {
            n133 = Unbundle By Name(w359) -> ("Folders"=w358:T9, "PackageNames"=w353:string[])
            n134 = for {
              tunnel: w358 -> [w367] mode=indexing
              shift-right: [w368] -> w356
              shift-left: w354 -> [w366]
              shift-right: [w369] -> w357
              shift-left: w360 -> [w370]
              tunnel: w353 -> [w363]
              n135 = Unbundle By Name(w367) -> ("PackageNode"=w365:refnum<class "PackageNode.lvclass">, "Foldername"=w364:string)
              n136 = Search 1D Array(1D array=w363, element=w364) -> (index of element=w362:i32)  [unwired: 1 in]
              n137 = case shown="0, Default" w362 {
                tunnel: w370 -> [w372 w378]
                tunnel: [w372 w377] -> w369
                tunnel: [w371 w376] -> w368
                tunnel: w366 -> [w371 w374]
                tunnel: w365 -> [_ w373]
                frame 0, Default {
                }
                frame -1 {
                  n138 = call-dynamic "addNode.vi"("reference"=w378, "node"=w373, "point"=T6 {"x"=nan, "y"=nan}, "error in (no error)"=w374) -> ("reference out"=w377:refnum<class "Graph.lvclass">, "error out"=w376:errorcluster)  [unwired: 14 in]
                }
              }
            }
            n139 = call-dynamic "layout.vi"("reference"=w357, "error in (no error)"=w356) -> ("error out"=w355:errorcluster)  [unwired: 16 in, 1 out]
          }
        }
        n140 = Unbundle By Name(w40) -> ("status"=w39:bool)
        n141 = Equal?(x=w38, y="Exit") -> (x = y?=w36:bool)
        n142 = Or(x=w36, y=w39) -> (x .or. y?=w35:bool)
      }
    }
    frame Error {
    }
  }
  n143 = call <resource>:"ContextHelp_LeavingDialog.vi"("error in (no error)"=w12) -> ("error out"=w8:errorcluster)  [unwired: 18 out]
  n144 = property class="VI"(error in=w12, "Front Panel.Open"=FALSE ("Front Panel Window:Open")) -> (error out=→"error out":errorcluster)  [unwired: 1 in, 1 out]
  n145 = call <resource>:"UMLEditor ControlBusyDialog.vi"("error in (no error)"=w8, "Action(SendStatusMessage)"=UMLEditor_BusyDialogAction."Close" ("Action")) -> ()  [unwired: 2 in, 16 out]
